vi "nominal convert results recursor.vi"(7 "hierarchy path":string, 11 "property bag":refnum<k7>) -> (1 "numerics":T1[](array[typedef]), 2 "strings":T2(array[cluster]), 3 "Report Text":string)   [LabVIEW 2020, in "nominal teststand model sequence support.lvlib"]
uses:
  nominal teststand model sequence support.lvlib
  nominal numeric result collection.ctl
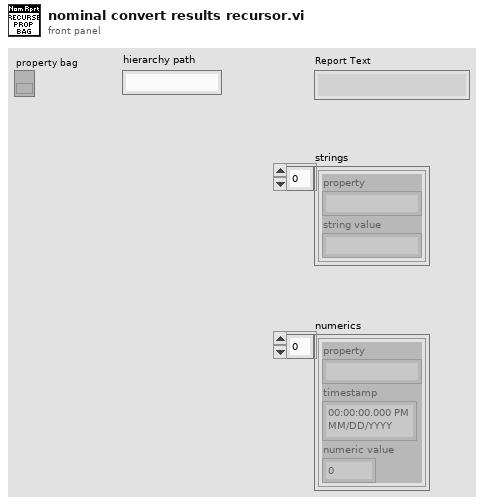
[diagram p1: front panel]
types:
  T1 = typedef "nominal teststand model sequence support.lvlib/nominal numeric result collection.ctl" = cluster{"property":string, "timestamp":timestamp, "numeric value":dbl}
  T2 = cluster{"property":string, "string value":string}[]
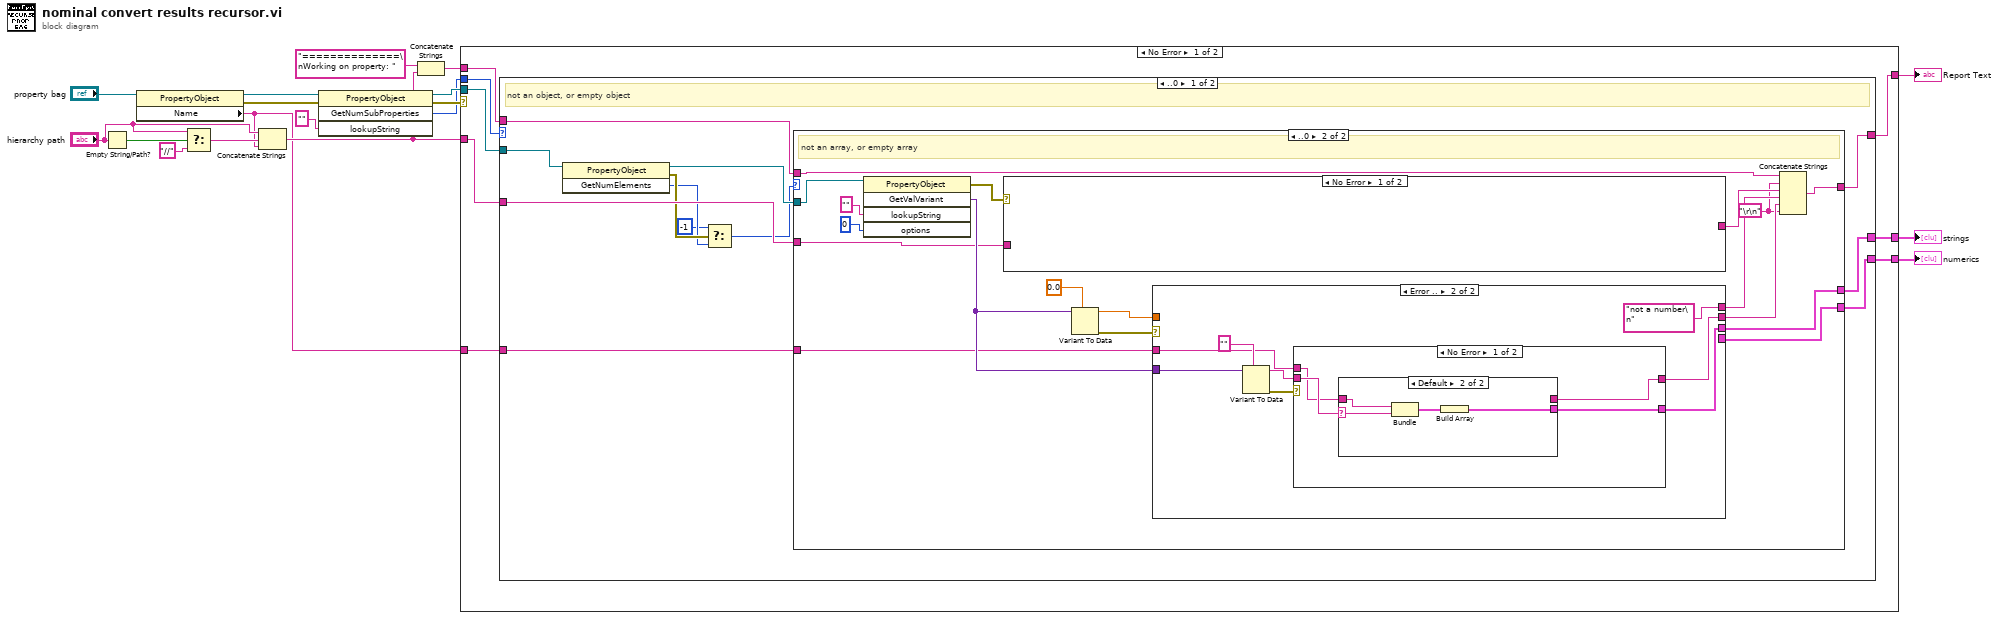
[diagram p0: block diagram]
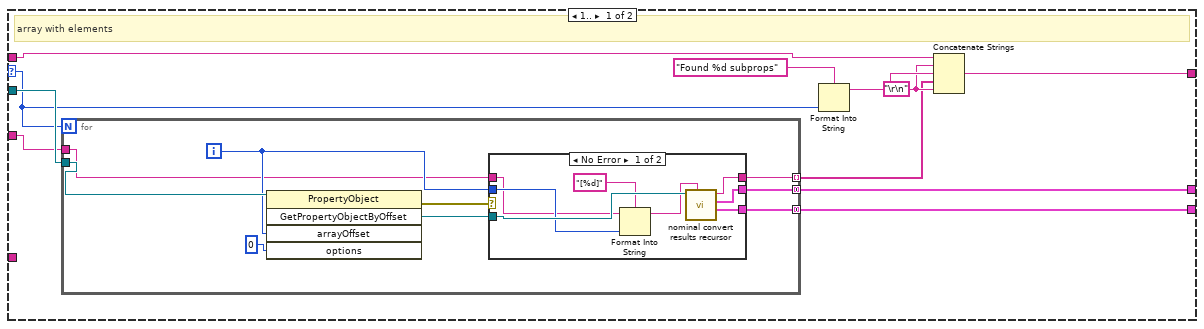
[diagram p2: hidden frame]
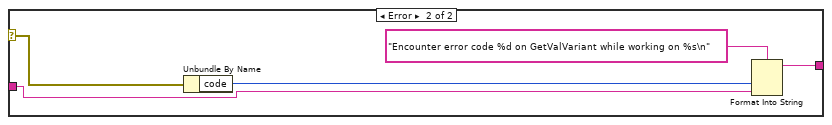
[diagram p4: hidden frame]
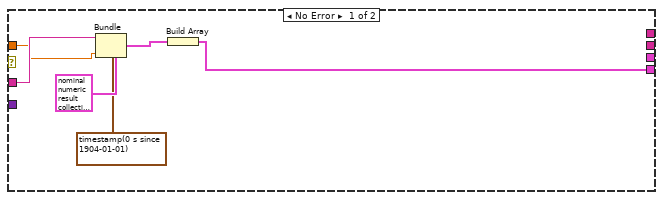
[diagram p5: hidden frame]
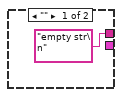
[diagram p6: hidden frame]
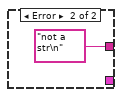
[diagram p7: hidden frame]
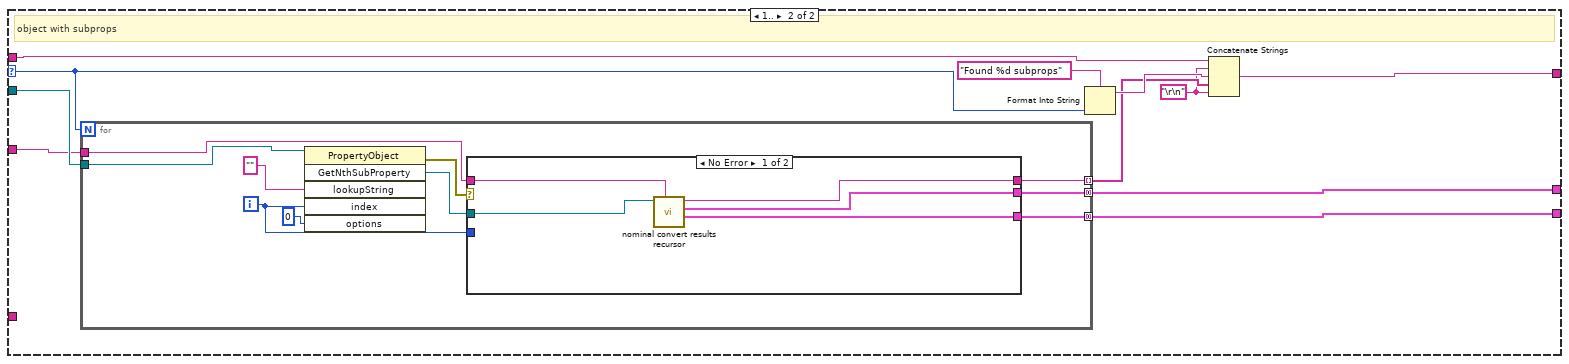
[diagram p8: hidden frame]
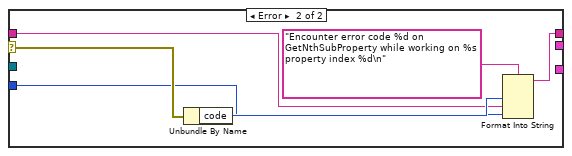
[diagram p9: hidden frame]
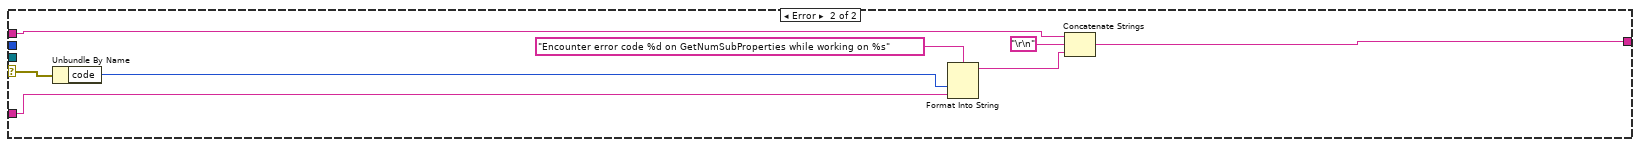
[diagram p10: hidden frame]
diagram:
  n1 = Empty String/Path?(string/path="hierarchy path") -> (empty?=w5:bool)
  n2 = property class="PropertyObject"(reference="property bag") -> (reference out=w10:refnum<k7>, error out=w11:errorcluster, "Name"=w1:string)  [unwired: 1 in]
  n3 = Select(t="hierarchy path", s=w5, f="//" ("string")) -> (s? t:f=w2:string)
  n4 = Concatenate Strings("hierarchy path", w2, w1) -> (w6:string)
  n5 = invoke class="PropertyObject" method="GetNumSubProperties"(reference=w10, error in=w11, "lookupString"="") -> (reference out=w14:refnum<k7>, error out=w15:errorcluster, "GetNumSubProperties"=w13:i32)  [unwired: 1 in, 1 out]
  n6 = Concatenate Strings("==============\nWorking on property: " ("string"), w6) -> (w8:string)
  n7 = case shown="No Error" w15 {
    selector: w15 -> [_ w147]
    tunnel: w14 -> [w26 _]
    tunnel: w13 -> [w25 _]
    tunnel: [w24 _] -> w17
    tunnel: [w23 _] -> w18
    tunnel: w6 -> [w22 w148]
    tunnel: w8 -> [w21 w153]
    tunnel: [w20 w151] -> w7
    tunnel: w1 -> [w19 _]
    frame No Error {
      n8 = case shown="..0" w25 {
        selector: w25 -> [_ w121]
        tunnel: w26 -> [w33 w124]
        tunnel: [w38 w116] -> w24
        tunnel: [w37 w117] -> w23
        tunnel: w22 -> [w36 w114]
        tunnel: w21 -> [w34 w123]
        tunnel: [w35 w119] -> w20
        tunnel: w19 -> [w27 _]
        frame ..0 {
          # "not an object, or empty object"
          n9 = invoke class="PropertyObject" method="GetNumElements"(reference=w33) -> (reference out=w32:refnum<k7>, error out=w31:errorcluster, "GetNumElements"=w30:i32)  [unwired: 2 in]
          n10 = Select(t=-1, s=w31, f=w30) -> (s? t:f=w28:i32)
          n11 = case shown="..0" w28 {
            selector: w28 -> [w42 _]
            tunnel: [w39 w81] -> w38
            tunnel: [w40 w79] -> w37
            tunnel: w36 -> [w48 w75]
            tunnel: [w44 w73] -> w35
            tunnel: w34 -> [w43 w70]
            tunnel: w32 -> [w49 w68]
            tunnel: w27 -> [_ w67]
            frame 1.. {
              w45 = "\r\n"
              # "array with elements"
              n12 = for {
                N: w42 -> [_]
                tunnel: w49 -> [w58]
                tunnel: w48 -> [w53]
                tunnel: [w52] -> w41 mode=indexing
                tunnel: [w51] -> w40 mode=concatenating
                tunnel: [w50] -> w39 mode=concatenating
                i -> [w54]
                n13 = invoke class="PropertyObject" method="GetPropertyObjectByOffset"(reference=w58, "arrayOffset"=w54, "options"=0) -> (error out=w55:errorcluster, "GetPropertyObjectByOffset"=w56:refnum<k7>)  [unwired: 2 in, 3 out]
                n14 = case shown="No Error" w55 {
                  tunnel: w56 -> [w66 _]
                  tunnel: w54 -> [w64 _]
                  tunnel: w53 -> [w63 _]
                  tunnel: [w61 _] -> w52
                  tunnel: [w60 _] -> w51
                  tunnel: [w59 _] -> w50
                  frame No Error {
                    n15 = Format Into String(format string="[%d]", initial string=w63, w64) -> (resulting string=w65:string)  [unwired: 1 in, 1 out]
                    n16 = call "nominal convert results recursor.vi"("hierarchy path"=w65, "property bag"=w66) -> ("numerics"=w59:T1[], "strings"=w60:T2, "Report Text"=w61:string)  [unwired: 7 in]
                  }
                  frame Error {
                  }
                }
              }
              n17 = Format Into String(format string="Found %d subprops", w42) -> (resulting string=w47:string)  [unwired: 2 in, 1 out]
              n18 = Concatenate Strings(w43, w45, w47, w41, w45) -> (w44:string)
            }
            frame ..0 {
              w69 = "\r\n"
              # "not an array, or empty array"
              n19 = invoke class="PropertyObject" method="GetValVariant"(reference=w68, "lookupString"="", "options"=0) -> (error out=w76:errorcluster, "GetValVariant"=w78:variant)  [unwired: 2 in, 3 out]
              n20 = case shown="No Error" w76 {
                selector: w76 -> [_ w88]
                tunnel: w75 -> [_ w85]
                tunnel: [_ w86] -> w71
                frame No Error {
                }
                frame Error {
                  n21 = Unbundle By Name(w88) -> ("code"=w87:i32)
                  n22 = Format Into String(format string="Encounter error code %d on GetValVariant while working on %s\n", w87, w85) -> (resulting string=w86:string)  [unwired: 2 in, 1 out]
                }
              }
              n23 = Variant To Data(type=0.0, Variant=w78) -> (data=w82:dbl, error out=w80:errorcluster)  [unwired: 1 in]
              n24 = case shown="Error .." w80 {
                tunnel: w82 -> [w91 _]
                tunnel: [w95 _] -> w81
                tunnel: [_ w103] -> w79
                tunnel: w78 -> [_ w102]
                tunnel: w67 -> [w93 w98]
                tunnel: [_ "not a number\n" ("string")] -> w74
                tunnel: [_ w96] -> w72
                frame No Error {
                  n25 = Bundle(cluster=T1 {"property"="", "timestamp"=timestamp(0 s since 1904-01-01), "numeric value"=0.0} ("Cluster"), "property"=w93, "timestamp"=timestamp(0 s since 1904-01-01), "numeric value"=w91) -> (w94:T1)
                  n26 = Build Array(w94) -> (w95:T1[])
                }
                frame Error {
                  n27 = Variant To Data(type="", Variant=w102) -> (data=w100:string, error out=w99:errorcluster)  [unwired: 1 in]
                  n28 = case shown="No Error" w99 {
                    tunnel: [w107 _] -> w103
                    tunnel: w100 -> [w106 _]
                    tunnel: w98 -> [w105 _]
                    tunnel: [w104 "not a str\n" ("string")] -> w96
                    frame No Error {
                      n29 = case shown="Default" w106 {
                        selector: w106 -> [_ w111]
                        tunnel: [_ w112] -> w107
                        tunnel: w105 -> [_ w109]
                        tunnel: ["empty str\n" ("string") _] -> w104
                        frame "" {
                        }
                        frame Default {
                          n30 = Bundle("Name"=w109, w111) -> (w110:cluster{"Name":string, string})  [unwired: 1 in]
                          n31 = Build Array(w110) -> (w112:cluster{"Name":string, string}[])
                        }
                      }
                    }
                    frame Error {
                    }
                  }
                }
              }
              n32 = Concatenate Strings(w70, w69, w71, w74, w72, w69) -> (w73:string)
            }
          }
        }
        frame 1.. {
          w115 = "\r\n"
          # "object with subprops"
          n33 = for {
            N: w121 -> [_]
            tunnel: w124 -> [w134]
            tunnel: [w129] -> w118 mode=indexing
            tunnel: w114 -> [w125]
            tunnel: [w127] -> w117 mode=concatenating
            tunnel: [w126] -> w116 mode=concatenating
            i -> [w128]
            n34 = invoke class="PropertyObject" method="GetNthSubProperty"(reference=w134, "lookupString"="", "index"=w128, "options"=0) -> (error out=w130:errorcluster, "GetNthSubProperty"=w131:refnum<k7>)  [unwired: 2 in, 4 out]
            n35 = case shown="No Error" w130 {
              selector: w130 -> [_ w143]
              tunnel: w131 -> [w139 _]
              tunnel: [w138 w144] -> w129
              tunnel: w128 -> [_ w141]
              tunnel: [w135 _] -> w127
              tunnel: [w136 _] -> w126
              tunnel: w125 -> [w137 w140]
              frame No Error {
                n36 = call "nominal convert results recursor.vi"("hierarchy path"=w137, "property bag"=w139) -> ("numerics"=w136:T1[], "strings"=w135:T2, "Report Text"=w138:string)  [unwired: 7 in]
              }
              frame Error {
                n37 = Unbundle By Name(w143) -> ("code"=w142:i32)
                n38 = Format Into String(format string="Encounter error code %d on GetNthSubProperty while working on %s property index %d\n", w142, w140, w141) -> (resulting string=w144:string)  [unwired: 2 in, 1 out]
              }
            }
          }
          n39 = Format Into String(format string="Found %d subprops", w121) -> (resulting string=w122:string)  [unwired: 2 in, 1 out]
          n40 = Concatenate Strings(w123, w115, w122, w118, w115) -> (w119:string)
        }
      }
    }
    frame Error {
      n41 = Unbundle By Name(w147) -> ("code"=w146:i32)
      n42 = Format Into String(format string="Encounter error code %d on GetNumSubProperties while working on %s", w146, w148) -> (resulting string=w149:string)  [unwired: 2 in, 1 out]
      n43 = Concatenate Strings(w153, "\r\n", w149) -> (w151:string)
    }
  }
  "Report Text" <- w7
  "strings" <- w18
  "numerics" <- w17
